vi "MINIPROJECTFINAL (1).vi"() -> ()   [LabVIEW 2022 SP3]
panel:
  out "COST 6":i32
  out "COST 5":i32
  out "COST 4":i32
  out "COST 3":i32
  out "COST 2":i32
  out "COST 1":i32
  out "TIME 6":i32
  out "TIME 5":i32
  out "TIME 4":i32
  out "TIME 3":i32
  out "TIME 2":i32
  out "TIME 1":i32
  out "PARKING SLOT 6":bool
  out "PARKING SLOT 5":bool
  out "PARKING SLOT 4":bool
  out "PARKING SLOT 3":bool
  out "PARKING SLOT 2":bool
  out "PARKING SLOT 1":bool
  in  "CAR ENTRY":bool
  out "SLOT 6":bool
  out "SLOT 5":bool
  out "SLOT 4":bool
  out "SLOT 3":bool
  out "SLOT 2":bool
  out "SLOT 1":bool
  # "E\nN\nT\nR\nY"
  # "E\nX\nI\nT"
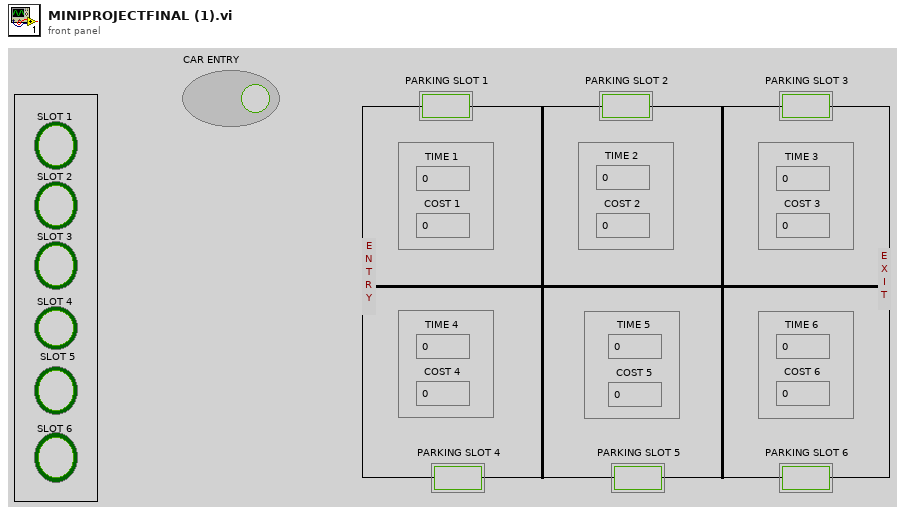
[diagram p1: front panel]
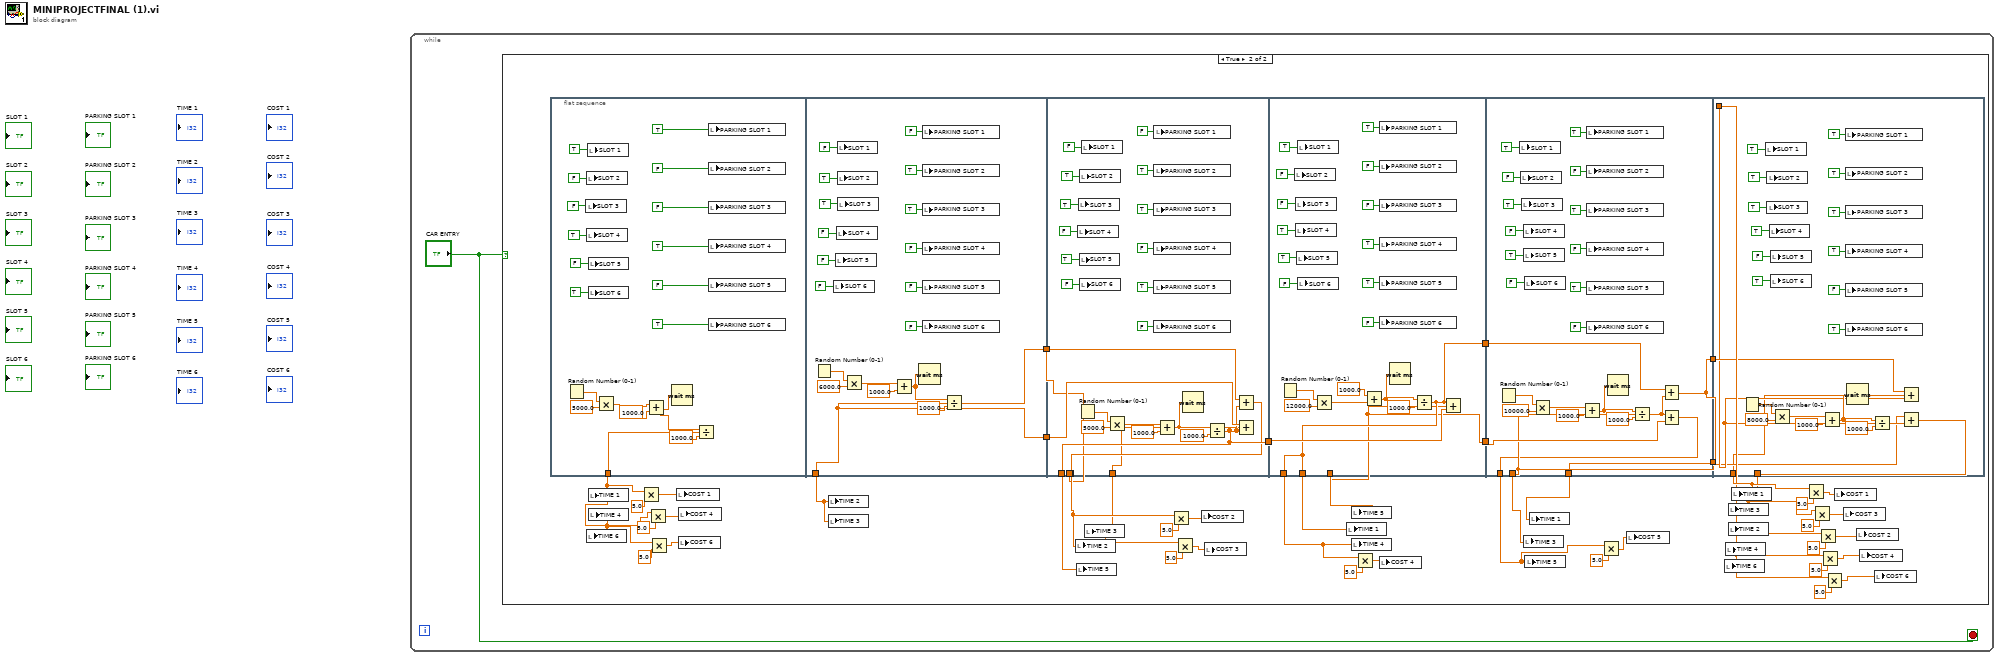
[diagram p0: block diagram]
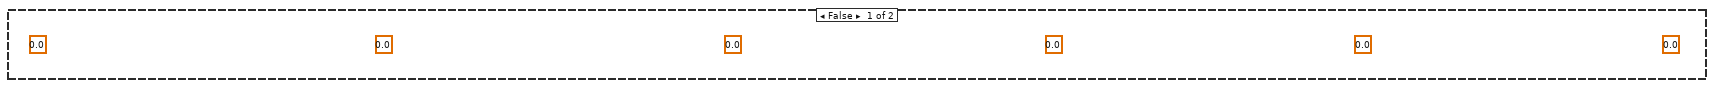
[diagram p2: hidden frame]
diagram:
  n1 = while {
    stop <- "CAR ENTRY" stop-if-true
    n2 = case shown="True" "CAR ENTRY" {
      frame False {
        (unwired) 0.0
        (unwired) 0.0
        (unwired) 0.0
        (unwired) 0.0
        (unwired) 0.0
        (unwired) 0.0
      }
      frame True {
        n3 = flat-sequence {
          tunnel: [w47] -> w29
          tunnel: [w66] -> w46
          tunnel: [w66] -> w37
          tunnel: [w66] -> w36
          tunnel: [w88] -> w44
          tunnel: [w88] -> w43
          tunnel: w37 -> [w85]
          tunnel: w36 -> [w89]
          tunnel: [w87] -> w25
          tunnel: [w86] -> w24
          tunnel: [w85] -> _
          tunnel: w43 -> [w110]
          tunnel: [w109] -> w42
          tunnel: [w109] -> w19
          tunnel: [w108] -> w41
          tunnel: [w109] -> w40
          tunnel: [w108] -> w35
          tunnel: [w132] -> w45
          tunnel: w41 -> [w134]
          tunnel: w40 -> [w133]
          tunnel: [w131] -> w39
          tunnel: [w132] -> w38
          tunnel: [w131] -> w34
          tunnel: [w130] -> w16
          tunnel: [w155] -> w2
          tunnel: w39 -> [w156]
          tunnel: w38 -> [w154]
          tunnel: [w153] -> w6
          tunnel: [w152] -> w9
          frame #0 {
            n4 = Random Number (0-1)() -> (number: 0 to 1=w60:dbl)
            n5 = local write "SLOT 3"(FALSE ("SLOT 3")) -> ()
            n6 = local write "SLOT 2"(FALSE ("SLOT 2")) -> ()
            n7 = local write "SLOT 4"(TRUE ("SLOT 4")) -> ()
            n8 = local write "SLOT 1"(TRUE ("SLOT 1")) -> ()
            n9 = local write "SLOT 5"(FALSE ("SLOT 5")) -> ()
            n10 = local write "SLOT 6"(TRUE ("SLOT 6")) -> ()
            n11 = Multiply(x=w60, y=5000.0) -> (x*y=w58:dbl)
            n12 = Add(x=w58, y=1000.0) -> (x+y=w48:dbl)
            n13 = Wait (ms)(milliseconds to wait=w48) -> ()  [unwired: 1 out]
            n14 = Divide(x=w48, y=1000.0) -> (x/y=w47:dbl)
            n15 = local write "PARKING SLOT 1"(TRUE ("PARKING SLOT 1")) -> ()
            n16 = local write "PARKING SLOT 2"(FALSE ("PARKING SLOT 2")) -> ()
            n17 = local write "PARKING SLOT 3"(FALSE ("PARKING SLOT 3")) -> ()
            n18 = local write "PARKING SLOT 4"(TRUE ("PARKING SLOT 4")) -> ()
            n19 = local write "PARKING SLOT 5"(FALSE ("PARKING SLOT 5")) -> ()
            n20 = local write "PARKING SLOT 6"(TRUE ("PARKING SLOT 6")) -> ()
          }
          frame #1 {
            n21 = Random Number (0-1)() -> (number: 0 to 1=w77:dbl)
            n22 = local write "SLOT 6"(FALSE ("SLOT 6")) -> ()
            n23 = local write "SLOT 5"(FALSE ("SLOT 5")) -> ()
            n24 = local write "SLOT 4"(FALSE ("SLOT 4")) -> ()
            n25 = local write "SLOT 1"(FALSE ("SLOT 1")) -> ()
            n26 = local write "SLOT 2"(TRUE ("SLOT 2")) -> ()
            n27 = local write "SLOT 3"(TRUE ("SLOT 3")) -> ()
            n28 = Multiply(x=w77, y=6000.0) -> (x*y=w78:dbl)
            n29 = Add(x=w78, y=1000.0) -> (x+y=w67:dbl)
            n30 = Wait (ms)(milliseconds to wait=w67) -> ()  [unwired: 1 out]
            n31 = local write "PARKING SLOT 1"(FALSE ("PARKING SLOT 1")) -> ()
            n32 = local write "PARKING SLOT 2"(TRUE ("PARKING SLOT 2")) -> ()
            n33 = local write "PARKING SLOT 3"(TRUE ("PARKING SLOT 3")) -> ()
            n34 = local write "PARKING SLOT 4"(FALSE ("PARKING SLOT 4")) -> ()
            n35 = local write "PARKING SLOT 5"(FALSE ("PARKING SLOT 5")) -> ()
            n36 = local write "PARKING SLOT 6"(FALSE ("PARKING SLOT 6")) -> ()
            n37 = Divide(x=w67, y=1000.0) -> (x/y=w66:dbl)
          }
          frame #2 {
            n38 = Random Number (0-1)() -> (number: 0 to 1=w100:dbl)
            n39 = local write "SLOT 4"(FALSE ("SLOT 4")) -> ()
            n40 = local write "SLOT 3"(TRUE ("SLOT 3")) -> ()
            n41 = local write "SLOT 5"(TRUE ("SLOT 5")) -> ()
            n42 = local write "SLOT 2"(TRUE ("SLOT 2")) -> ()
            n43 = local write "SLOT 6"(FALSE ("SLOT 6")) -> ()
            n44 = local write "SLOT 1"(FALSE ("SLOT 1")) -> ()
            n45 = Multiply(x=w100, y=5000.0) -> (x*y=w101:dbl)
            n46 = local write "PARKING SLOT 1"(FALSE ("PARKING SLOT 1")) -> ()
            n47 = local write "PARKING SLOT 2"(TRUE ("PARKING SLOT 2")) -> ()
            n48 = local write "PARKING SLOT 3"(TRUE ("PARKING SLOT 3")) -> ()
            n49 = local write "PARKING SLOT 4"(FALSE ("PARKING SLOT 4")) -> ()
            n50 = local write "PARKING SLOT 5"(TRUE ("PARKING SLOT 5")) -> ()
            n51 = local write "PARKING SLOT 6"(FALSE ("PARKING SLOT 6")) -> ()
            n52 = Add(x=w101, y=1000.0) -> (x+y=w90:dbl)
            n53 = Wait (ms)(milliseconds to wait=w90) -> ()  [unwired: 1 out]
            n54 = Divide(x=w90, y=1000.0) -> (x/y=w88:dbl)
            n55 = Add(x=w85, y=w88) -> (x+y=w87:dbl)
            n56 = Add(x=w89, y=w88) -> (x+y=w86:dbl)
          }
          frame #3 {
            n57 = Random Number (0-1)() -> (number: 0 to 1=w121:dbl)
            n58 = local write "SLOT 2"(FALSE ("SLOT 2")) -> ()
            n59 = local write "SLOT 3"(FALSE ("SLOT 3")) -> ()
            n60 = local write "SLOT 4"(TRUE ("SLOT 4")) -> ()
            n61 = local write "SLOT 5"(TRUE ("SLOT 5")) -> ()
            n62 = local write "SLOT 1"(TRUE ("SLOT 1")) -> ()
            n63 = local write "SLOT 6"(FALSE ("SLOT 6")) -> ()
            n64 = Multiply(x=w121, y=12000.0) -> (x*y=w120:dbl)
            n65 = Add(x=1000.0, y=w120) -> (x+y=w111:dbl)
            n66 = local write "PARKING SLOT 1"(TRUE ("PARKING SLOT 1")) -> ()
            n67 = local write "PARKING SLOT 2"(FALSE ("PARKING SLOT 2")) -> ()
            n68 = local write "PARKING SLOT 3"(FALSE ("PARKING SLOT 3")) -> ()
            n69 = local write "PARKING SLOT 4"(TRUE ("PARKING SLOT 4")) -> ()
            n70 = local write "PARKING SLOT 5"(TRUE ("PARKING SLOT 5")) -> ()
            n71 = local write "PARKING SLOT 6"(FALSE ("PARKING SLOT 6")) -> ()
            n72 = Wait (ms)(milliseconds to wait=w111) -> ()  [unwired: 1 out]
            n73 = Divide(x=w111, y=1000.0) -> (x/y=w109:dbl)
            n74 = Add(x=w109, y=w110) -> (x+y=w108:dbl)
          }
          frame #4 {
            n75 = Random Number (0-1)() -> (number: 0 to 1=w129:dbl)
            n76 = local write "SLOT 1"(TRUE ("SLOT 1")) -> ()
            n77 = local write "SLOT 2"(FALSE ("SLOT 2")) -> ()
            n78 = local write "SLOT 3"(TRUE ("SLOT 3")) -> ()
            n79 = local write "SLOT 4"(FALSE ("SLOT 4")) -> ()
            n80 = local write "SLOT 5"(TRUE ("SLOT 5")) -> ()
            n81 = local write "SLOT 6"(FALSE ("SLOT 6")) -> ()
            n82 = Multiply(x=w129, y=10000.0) -> (x*y=w144:dbl)
            n83 = Add(x=w144, y=1000.0) -> (x+y=w135:dbl)
            n84 = local write "PARKING SLOT 1"(TRUE ("PARKING SLOT 1")) -> ()
            n85 = local write "PARKING SLOT 2"(FALSE ("PARKING SLOT 2")) -> ()
            n86 = local write "PARKING SLOT 3"(TRUE ("PARKING SLOT 3")) -> ()
            n87 = local write "PARKING SLOT 4"(FALSE ("PARKING SLOT 4")) -> ()
            n88 = local write "PARKING SLOT 5"(TRUE ("PARKING SLOT 5")) -> ()
            n89 = local write "PARKING SLOT 6"(FALSE ("PARKING SLOT 6")) -> ()
            n90 = Wait (ms)(milliseconds to wait=w135) -> ()  [unwired: 1 out]
            n91 = Divide(x=w135, y=1000.0) -> (x/y=w132:dbl)
            n92 = Add(x=w133, y=w132) -> (x+y=w131:dbl)
            n93 = Add(x=w132, y=w134) -> (x+y=w130:dbl)
          }
          frame #5 {
            n94 = Random Number (0-1)() -> (number: 0 to 1=w167:dbl)
            n95 = local write "SLOT 1"(TRUE ("SLOT 1")) -> ()
            n96 = local write "SLOT 2"(TRUE ("SLOT 2")) -> ()
            n97 = local write "SLOT 3"(TRUE ("SLOT 3")) -> ()
            n98 = local write "SLOT 4"(TRUE ("SLOT 4")) -> ()
            n99 = local write "SLOT 5"(FALSE ("SLOT 5")) -> ()
            n100 = local write "SLOT 6"(TRUE ("SLOT 6")) -> ()
            n101 = Multiply(x=w167, y=8000.0) -> (x*y=w166:dbl)
            n102 = Add(x=w166, y=1000.0) -> (x+y=w157:dbl)
            n103 = local write "PARKING SLOT 1"(TRUE ("PARKING SLOT 1")) -> ()
            n104 = local write "PARKING SLOT 2"(TRUE ("PARKING SLOT 2")) -> ()
            n105 = local write "PARKING SLOT 3"(TRUE ("PARKING SLOT 3")) -> ()
            n106 = local write "PARKING SLOT 4"(TRUE ("PARKING SLOT 4")) -> ()
            n107 = local write "PARKING SLOT 5"(FALSE ("PARKING SLOT 5")) -> ()
            n108 = local write "PARKING SLOT 6"(TRUE ("PARKING SLOT 6")) -> ()
            n109 = Wait (ms)(milliseconds to wait=w157) -> ()  [unwired: 1 out]
            n110 = Divide(x=w157, y=1000.0) -> (x/y=w155:dbl)
            n111 = Add(x=w156, y=w155) -> (x+y=w152:dbl)
            n112 = Add(x=w154, y=w155) -> (x+y=w153:dbl)
          }
        }
        n113 = local write "TIME 6"(w29) -> ()
        n114 = local write "TIME 1"(w29) -> ()
        n115 = local write "TIME 4"(w29) -> ()
        n116 = Multiply(x=w29, y=5.0) -> (x*y=w32:dbl)
        n117 = Multiply(x=w29, y=5.0) -> (x*y=w28:dbl)
        n118 = Multiply(x=w29, y=5.0) -> (x*y=w27:dbl)
        n119 = local write "COST 1"(w32) -> ()
        n120 = local write "COST 6"(w27) -> ()
        n121 = local write "COST 4"(w28) -> ()
        n122 = local write "TIME 2"(w46) -> ()
        n123 = local write "TIME 3"(w46) -> ()
        n124 = local write "TIME 2"(w25) -> ()
        n125 = local write "TIME 5"(w44) -> ()
        n126 = local write "TIME 3"(w24) -> ()
        n127 = Multiply(x=w25, y=5.0) -> (x*y=w26:dbl)
        n128 = Multiply(x=w24, y=5.0) -> (x*y=w23:dbl)
        n129 = local write "COST 2"(w26) -> ()
        n130 = local write "COST 3"(w23) -> ()
        n131 = local write "TIME 1"(w42) -> ()
        n132 = local write "TIME 5"(w35) -> ()
        n133 = local write "TIME 4"(w19) -> ()
        n134 = Multiply(x=w19, y=5.0) -> (x*y=w18:dbl)
        n135 = local write "COST 4"(w18) -> ()
        n136 = local write "TIME 3"(w45) -> ()
        n137 = local write "TIME 5"(w16) -> ()
        n138 = local write "TIME 1"(w34) -> ()
        n139 = Multiply(x=w16, y=5.0) -> (x*y=w15:dbl)
        n140 = local write "COST 5"(w15) -> ()
        n141 = local write "TIME 6"(w2) -> ()
        n142 = local write "TIME 4"(w2) -> ()
        n143 = local write "TIME 3"(w6) -> ()
        n144 = local write "TIME 2"(w2) -> ()
        n145 = local write "TIME 1"(w9) -> ()
        n146 = Multiply(x=w9, y=5.0) -> (x*y=w8:dbl)
        n147 = Multiply(x=w6, y=5.0) -> (x*y=w7:dbl)
        n148 = Multiply(x=w2, y=5.0) -> (x*y=w5:dbl)
        n149 = Multiply(x=w2, y=5.0) -> (x*y=w4:dbl)
        n150 = Multiply(x=w2, y=5.0) -> (x*y=w3:dbl)
        n151 = local write "COST 1"(w8) -> ()
        n152 = local write "COST 3"(w7) -> ()
        n153 = local write "COST 2"(w5) -> ()
        n154 = local write "COST 4"(w4) -> ()
        n155 = local write "COST 6"(w3) -> ()
      }
    }
  }
